vi "lvmcp_termind.vi"() -> ()   [LabVIEW 2015]
panel:
  out "error out":errorcluster
  in  "reference":refnum<vi>
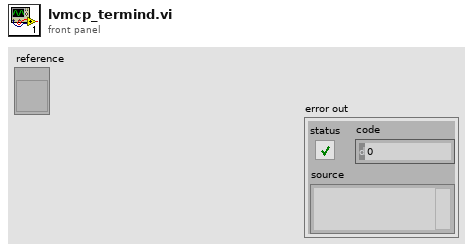
[diagram p1: front panel]
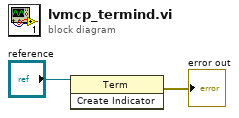
[diagram p0: block diagram]
diagram:
  n1 = invoke class="Term" method="Create Indicator"(reference="reference") -> (error out=→"error out":errorcluster)  [unwired: 2 in, 2 out]
